vi "AlliGator Mouse ID.vi"(8 "error in (no error)":errorcluster) -> (0 "error out":errorcluster, 1 "button info":T1, 2 "axis info":T2, 3 "Mouse ID":refnum<k1>)   [LabVIEW 2021, in "AlliGator GUI.lvlib"]
uses:
  AlliGator GUI.lvlib
  Globals, Variables, Constants/AlliGator Refnums List.ctl
panel:
  # "see the License on the block diagram (Ctrl+E or Window:Show Block Diagram)"
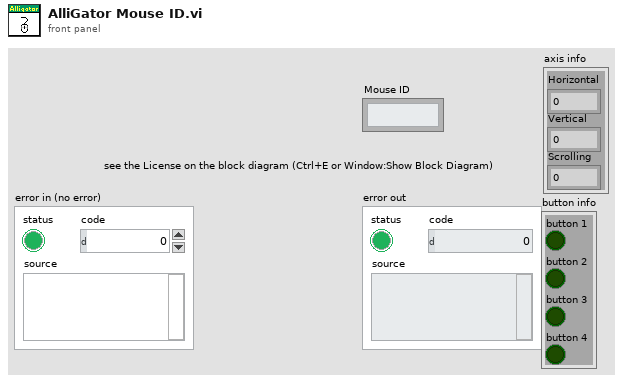
[diagram p1: front panel]
types:
  T1 = cluster{"button 1":bool, "button 2":bool, "button 3":bool, "button 4":bool}
  T2 = cluster{"Horizontal":i32, "Vertical":i32, "Scrolling":i32}
  T3 = typedef "AlliGator GUI.lvlib/AlliGator Refnums List.ctl" = enum16{"---------- AlliGator Control Refnums ----------", "AlliGator Tab Control Refnum", "Dataset Ctrl Refnums", "Image Histogram Ctrl Refnums", "Intensity Time Trace Ctrl Refnums", "Decay Graph Ctrl Refnums", "Decay Statistics Graph Ctrl Refnums", "Phasor Graph Ctrl Refnums", "Phasor Ratio Graph Ctrl Refnums", "Phasor Plot Ctrl Refnums", "Lifetime & Other Parameters Ctrl Refnums", "Decay Fit Parameter Map Ctrl Refnums", "Parameter Map Ctrl Refnums", "Other AlliGator Ctrl Refnums", "---------- AlliGator VI Refnums ----------", "AlliGator Refnum", "AlliGator Settings Refnum", "AlliGator Launcher Refnum", "---------- IO Device ID ----------", "Mouse ID", "Keyboard ID"}
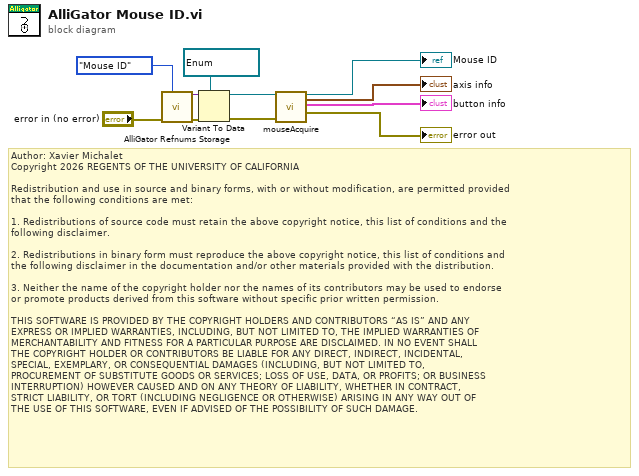
[diagram p0: block diagram]
diagram:
  w10 = refnum<k1> refnum items=["MOUSE"] ("device ID")
  # "Author: Xavier Michalet\nCopyright 2026 REGENTS OF THE UNIVERSITY OF CALIFORNIA\n\nRedistribution and use in source and binary forms, with or without modification, are permitted provided\nthat the following conditions are met:\n\n1. Redistributions of source code must retain the above copyright notice, this list of conditions and the\nfollowing disclaimer.\n\n2. Redistributions in binary form must reproduce the above copyright notice, this list of conditions and\nthe following disclaimer in the documentation and/or other materials provided with the distribution.\n\n3. Neither the name of the copyright holder nor the names of its contributors may be used to endorse \nor promote products derived from this software without specific prior written permission.\n\nTHIS SOFTWARE IS PROVIDED BY THE COPYRIGHT HOLDERS AND CONTRIBUTORS “AS IS” AND ANY \nEXPRESS OR IMPLIED WARRANTIES, INCLUDING, BUT NOT LIMITED TO, THE IMPLIED WARRANTIES OF\nMERCHANTABILITY AND FITNESS FOR A PARTICULAR PURPOSE ARE DISCLAIMED. IN NO EVENT SHALL\nTHE COPYRIGHT HOLDER OR CONTRIBUTORS BE LIABLE FOR ANY DIRECT, INDIRECT, INCIDENTAL, \nSPECIAL, EXEMPLARY, OR CONSEQUENTIAL DAMAGES (INCLUDING, BUT NOT LIMITED TO, \nPROCUREMENT OF SUBSTITUTE GOODS OR SERVICES; LOSS OF USE, DATA, OR PROFITS; OR BUSINESS\nINTERRUPTION) HOWEVER CAUSED AND ON ANY THEORY OF LIABILITY, WHETHER IN CONTRACT, \nSTRICT LIABILITY, OR TORT (INCLUDING NEGLIGENCE OR OTHERWISE) ARISING IN ANY WAY OUT OF\nTHE USE OF THIS SOFTWARE, EVEN IF ADVISED OF THE POSSIBILITY OF SUCH DAMAGE."
  n1 = call "AlliGator Refnums Storage.vi"("AlliGator Refnum List"=AlliGator_Refnums_List."Mouse ID", "Error In"="error in (no error)") -> ("Error Out"=w8:errorcluster, "Data out"=w9:variant)  [unwired: 8 in]
  n2 = Variant To Data(error in=w8, type=w10, Variant=w9) -> (data=w4:refnum<k1>, error out=w5:errorcluster)
  "error out" <- w5
  n3 = call <vilib>:"mouseAcquire.vi"("device ID"=w4, "error in (no error)"=w5) -> ("device ID"=→"Mouse ID":refnum<k1>, "axis info"=→"axis info":T2, "button info"=→"button info":T1)  [unwired: 14 in, 1 out]
